vi "Send.vi"(7 "VolatusAPI":refnum<class "VolatusAPI.lvclass">, 10 "Value":dbl, 11 "Numeric Command in":refnum<class "Numeric Command.lvclass">) -> (0 "error out":errorcluster)   [LabVIEW 2020, in "Volatus.lvlib" / "Numeric Command.lvclass"]
uses:
  Numeric Command.lvclass
  Numeric Command.lvclass/Numeric Command.ctl
  VolatusAPI/VolatusAPI.lvclass
  MessageQ/MessageQ.lvclass
  messages/CmdAnalog/Class/Msg.lvclass
  C:/dev/lv20CE/relink/lv-volatus/messages/CmdAnalog/Class/Msg.lvclass
  C:/dev/lv20CE/relink/lv-protoc/LV-Proto/Message/Message.lvclass
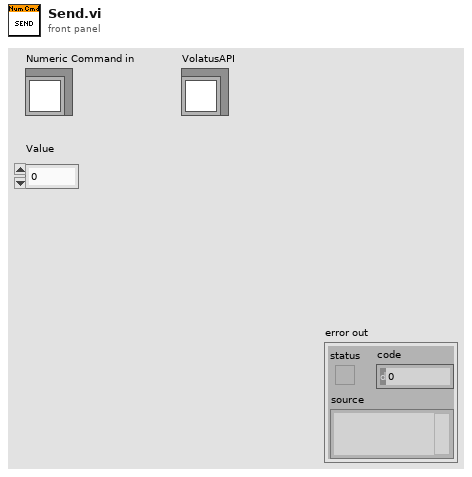
[diagram p1: front panel]
types:
  T1 = typedef "CmdAnalog.lvlib/Data.ctl" = cluster{"channel":string, "value":dbl}
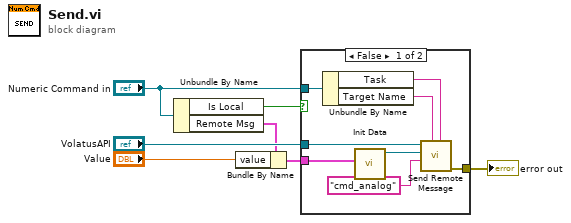
[diagram p0: block diagram]
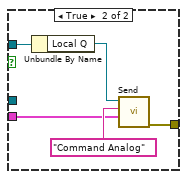
[diagram p2: hidden frame]
diagram:
  n1 = Unbundle By Name("Numeric Command in") -> ("Is Local"=w7:bool, "Remote Msg"=w5:T1)
  n2 = Bundle By Name(cluster=w5, "value"="Value") -> (w3:T1)
  n3 = case shown="False" w7 {
    tunnel: "VolatusAPI" -> [w15 _]
    tunnel: w3 -> [w14 w17]
    tunnel: "Numeric Command in" -> [w11 w20]
    tunnel: [w8 w16] -> w1
    frame False {
      n4 = Unbundle By Name(w11) -> ("Task"=w9:string, "Target Name"=w10:string)
      n5 = call "Init Data.vi"("Data"=w14) -> ("Msg out"=w13:refnum<class "Msg.lvclass">)  [unwired: 10 in]
      n6 = call "Send Remote Message.vi"("Target Task (None)"=w9, "Target Name"=w10, "Message Type"="cmd_analog", "Message"=w13, "VolatusAPI in"=w15) -> ("error out"=w8:errorcluster)  [unwired: 5 in, 1 out]
    }
    frame True {
      n7 = Unbundle By Name(w20) -> ("Local Q"=w19:refnum<class "MessageQ.lvclass">)
      n8 = call "Send.vi"("Data"=w17, "ID"="Command Analog", "MessageQ in"=w19) -> ("error out"=w16:errorcluster)  [unwired: 7 in, 1 out]
    }
  }
  "error out" <- w1
